vi "TDMS Initialization and Tag Formation_MS.vi"(8 "error in":errorcluster caption="エラー入力（エラーなし）", 10 "Raw data":dbl[](array[numeric]), 11 "A TDMS Pass":path) -> (0 "error out":errorcluster caption="エラー出力", 2 "Table Tag C":T1, 3 "A TDMSファイル出力":refnum<k34>)   [LabVIEW 2018]
panel:
  out "AC Table Tag":string[](array[string])
  out "AR Table Tag":string[](array[string])
  out "B Table Tag":string[](array[string])
  out "R Table Tag":string[](array[string])
  out "S Table Tag":string[](array[string])
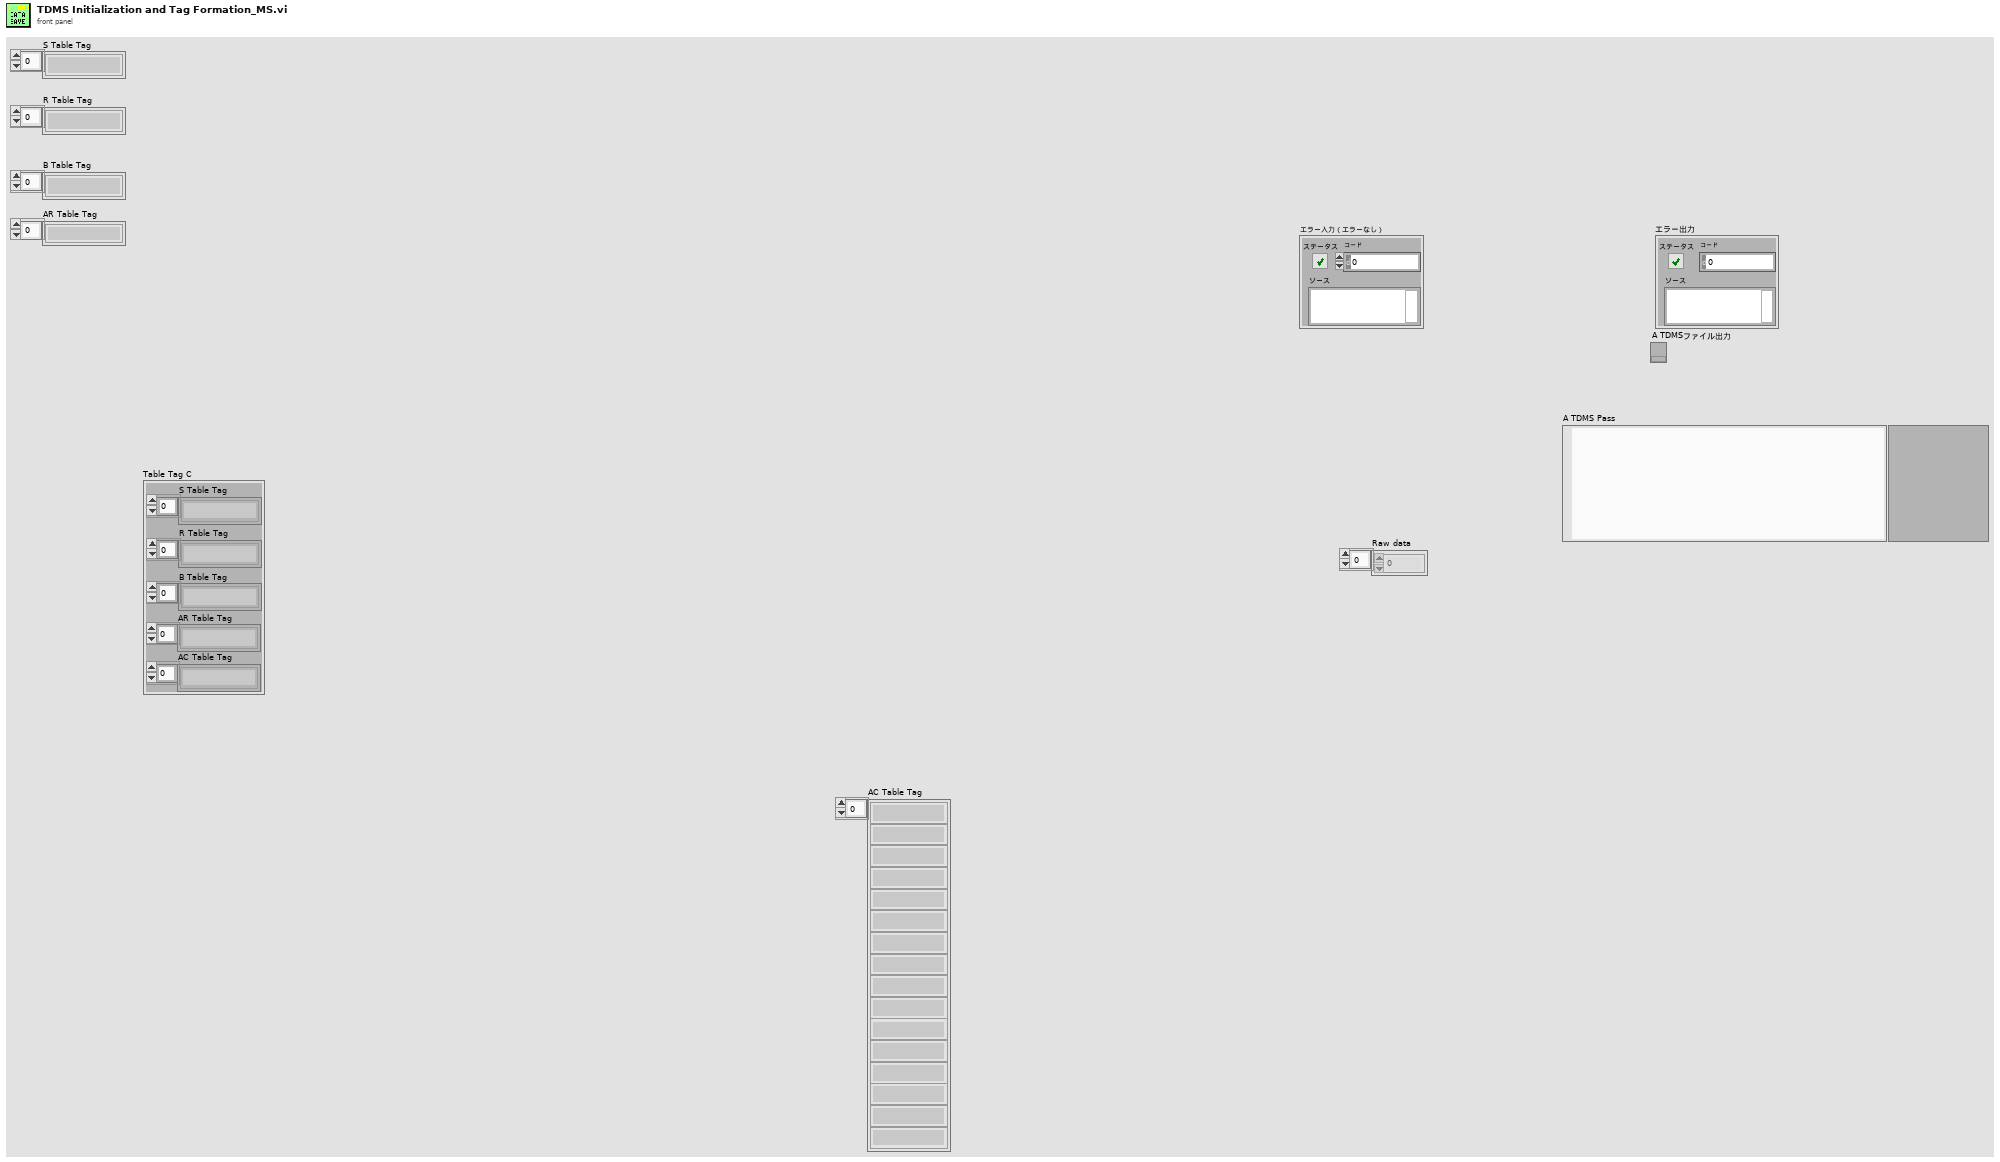
[diagram p1: front panel]
types:
  T1 = cluster{"S Table Tag":string[], "R Table Tag":string[], "B Table Tag":string[], "AR Table Tag":string[], "AC Table Tag":string[]}
  T2 = enum16{"open", "open or create", "create or replace", "create", "open (read-only)"}
  T3 = cluster{"行ヘッダ文字列[]":string[], "行ヘッダ文字列[]":string[], "行ヘッダ文字列[]":string[], "行ヘッダ文字列[]":string[], "行ヘッダ文字列[]":string[]}
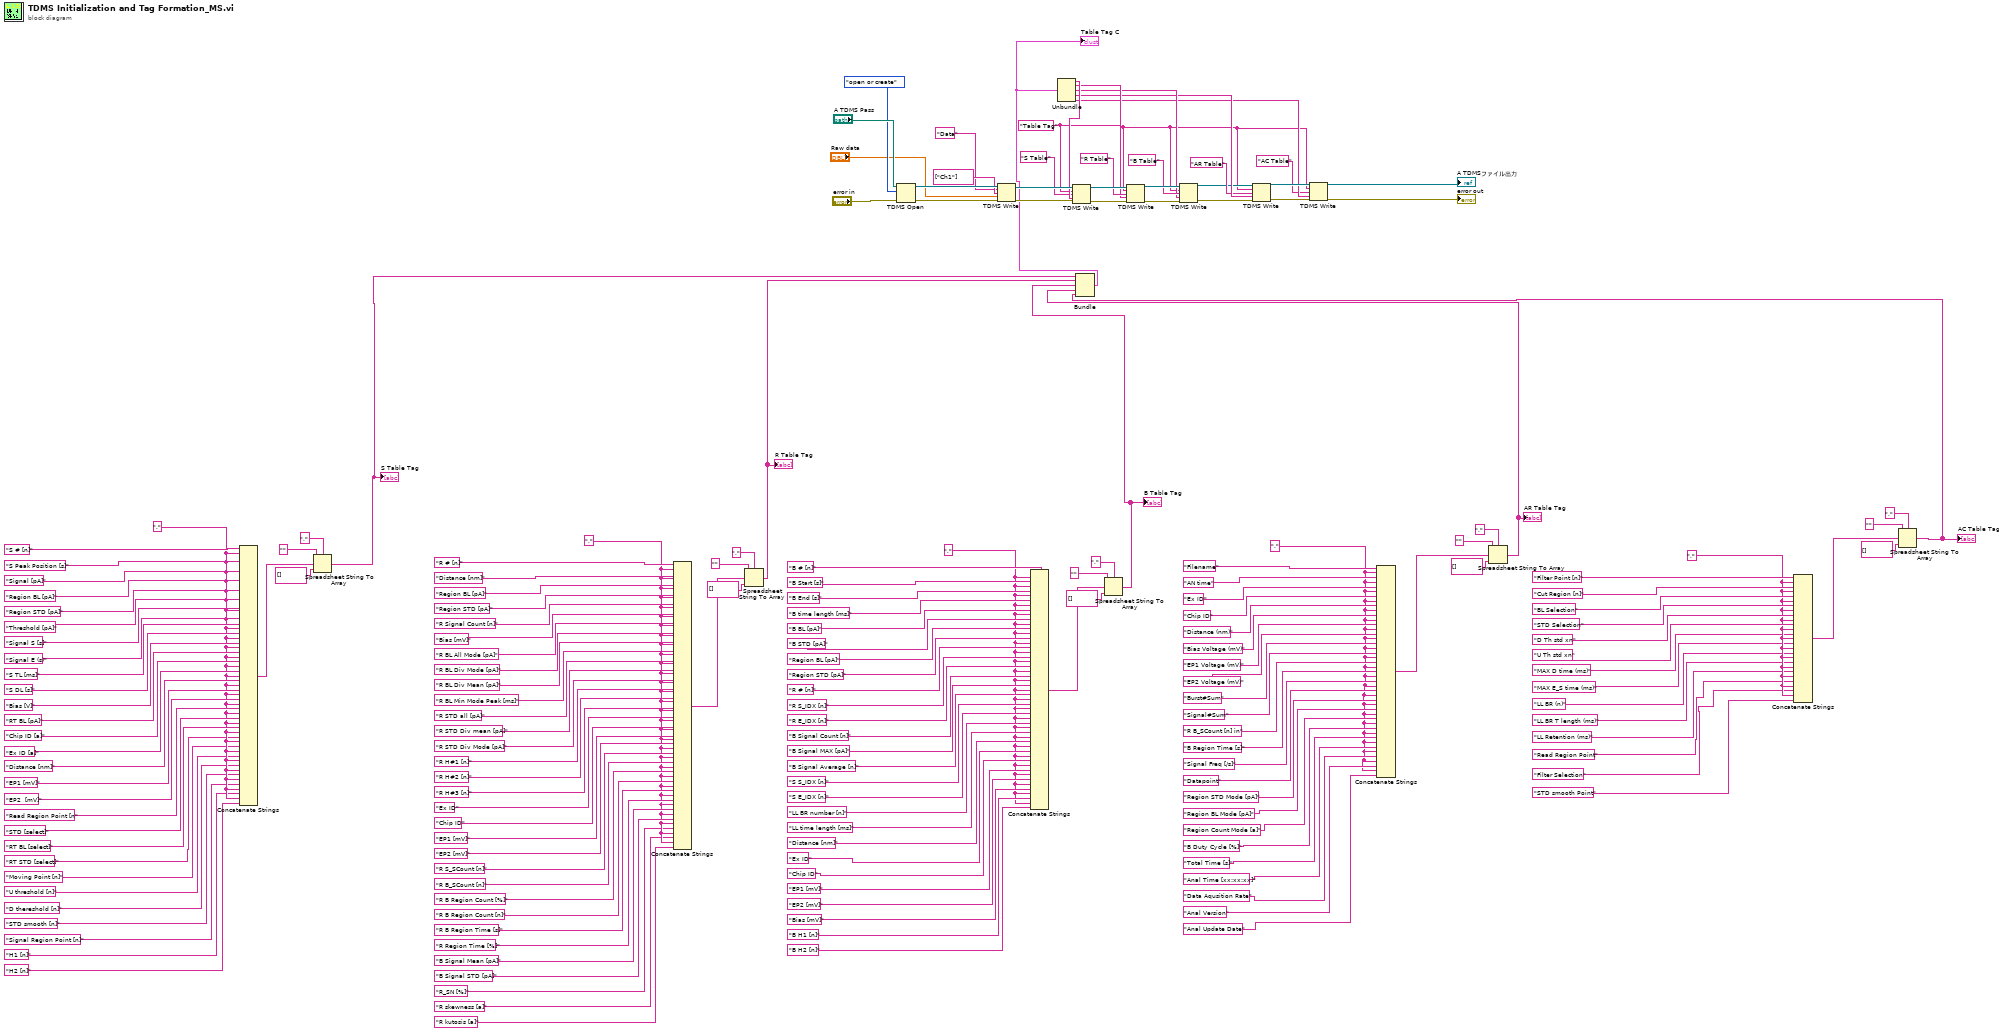
[diagram p0: block diagram]
diagram:
  w17 = "," ("デリミタ（タブ）")
  w37 = "," ("デリミタ（タブ）")
  w67 = "," ("デリミタ（タブ）")
  w105 = "," ("デリミタ（タブ）")
  w131 = "," ("デリミタ（タブ）")
  w1 = "Table Tag" ("グループ名入力（名称未設定）")
  n1 = Concatenate Strings("S # [n]" ("文字列"), w105, "S Peak Position [s]" ("文字列"), w105, "Signal [pA]" ("文字列"), w105, "Region BL [pA]" ("文字列"), w105, "Region STD [pA]" ("文字列"), w105, "Threshold [pA]" ("文字列"), w105, "Signal S [s]" ("文字列"), w105, "Signal E (s)" ("文字列"), w105, "S TL [ms]" ("文字列"), w105, "S DL [s]" ("文字列"), w105, "Bias [V]" ("文字列"), w105, "RT BL [pA]" ("文字列"), w105, "Chip ID [a]" ("文字列"), w105, "Ex ID [a]" ("文字列"), w105, "Distance [nm]" ("文字列"), w105, "EP1 [mV]" ("文字列"), w105, "EP2  [mV]" ("文字列"), w105, "Read Region Point [n" ("文字列"), w105, "STD [select]" ("文字列"), w105, "RT BL [select]" ("文字列"), w105, "RT STD [select]" ("文字列"), w105, "Moving Point [n]" ("文字列"), w105, "U threshold [n]" ("文字列"), w105, "D thereshold [n]" ("文字列"), w105, "STD smooth [n]" ("文字列"), w105, "Signal Region Point [n]" ("文字列"), w105, "H1 [n]" ("文字列"), w105, "H2 [n]" ("文字列")) -> (w125:string)
  n2 = Spreadsheet String To Array(delimiter (Tab)="," ("デリミタ（タブ）"), format string="" ("形式文字列"), spreadsheet string=w125, array type (2D Dbl)=string[] [] ("行ヘッダ文字列[]")) -> (array=w35:string[])
  "S Table Tag" <- w35
  n3 = Concatenate Strings("R # [n]" ("文字列"), w131, "Distance [nm]" ("文字列"), w131, "Region BL [pA]" ("文字列"), w131, "Region STD [pA]" ("文字列"), w131, "R Signal Count [n]" ("文字列"), w131, "Bias [mV]" ("文字列"), w131, "R BL All Mode [pA]" ("文字列"), w131, "R BL Div Mode [pA]" ("文字列"), w131, "R BL Div Mean [pA]" ("文字列"), w131, "R BL Min Mode Peak [ms]" ("文字列"), w131, "R STD all [pA]" ("文字列"), w131, "R STD Div mean [pA]" ("文字列"), w131, "R STD Div Mode [pA]" ("文字列"), w131, "R H#1 [n]" ("文字列"), w131, "R H#2 [n]" ("文字列"), w131, "R H#3 [n]" ("文字列"), w131, "Ex ID" ("文字列"), w131, "Chip ID" ("文字列"), w131, "EP1 [mV]" ("文字列"), w131, "EP2 [mV]" ("文字列"), w131, "R S_SCount [n]" ("文字列"), w131, "R B_SCount [n]" ("文字列"), w131, "R B Region Count [%]" ("文字列"), w131, "R B Region Count [n]" ("文字列"), w131, "R B Region Time [s]" ("文字列"), w131, "R Region Time [%]" ("文字列"), w131, "B Signal Mean [pA]" ("文字列"), w131, "B Signal STD [pA]" ("文字列"), w131, "R_SN [%]" ("文字列"), w131, "R skewness [a]" ("文字列"), w131, "R kutosis [a]" ("文字列")) -> (w160:string)
  n4 = Spreadsheet String To Array(delimiter (Tab)="," ("デリミタ（タブ）"), format string="" ("形式文字列"), spreadsheet string=w160, array type (2D Dbl)=string[] [] ("行ヘッダ文字列[]")) -> (array=w34:string[])
  "R Table Tag" <- w34
  n5 = TDMS Open(8:"error in", 10:T2."open or create" ("操作（0:open）"), 11:"A TDMS Pass") -> (0:w181:errorcluster, 3:w180:refnum<k34>)  [unwired: 4 in]
  n6 = TDMS Write(0:w180, 5:"Data" ("グループ名入力（名称未設定）"), 7:string[] ["Ch1"] ("チャンネル名入力（名称未設定）"), 9:"Raw data", 11:w181) -> (4:w175:refnum<k34>, 15:w176:errorcluster)  [unwired: 1 in, 2 out]
  n7 = Concatenate Strings("B # [n]" ("文字列"), w67, "B Start [s]" ("文字列"), w67, "B End [s]" ("文字列"), w67, "B time length [ms]" ("文字列"), w67, "B BL [pA]" ("文字列"), w67, "B STD [pA]" ("文字列"), w67, "Region BL [pA]" ("文字列"), w67, "Region STD [pA]" ("文字列"), w67, "R # [n]" ("文字列"), w67, "R S_IDX [n]" ("文字列"), w67, "R E_IDX [n]" ("文字列"), w67, "B Signal Count [n]" ("文字列"), w67, "B Signal MAX [pA]" ("文字列"), w67, "B Signal Average [n]" ("文字列"), w67, "S S_IDX [n]" ("文字列"), w67, "S E_IDX [n]" ("文字列"), w67, "LL BR number [n]" ("文字列"), w67, "LL time length [ms]" ("文字列"), w67, "Distance [nm]" ("文字列"), w67, "Ex ID" ("文字列"), w67, "Chip ID" ("文字列"), w67, "EP1 [mV]" ("文字列"), w67, "EP2 [mV]" ("文字列"), w67, "Bias [mV]" ("文字列"), w67, "B H1 [n]" ("文字列"), w67, "B H2 [n]" ("文字列")) -> (w92:string)
  n8 = Spreadsheet String To Array(delimiter (Tab)="," ("デリミタ（タブ）"), format string="" ("形式文字列"), spreadsheet string=w92, array type (2D Dbl)=string[] [] ("行ヘッダ文字列[]")) -> (array=w64:string[])
  "B Table Tag" <- w64
  n9 = Concatenate Strings("Filename" ("文字列"), w37, "AN time" ("文字列"), w37, "Ex ID" ("文字列"), w37, "Chip ID" ("文字列"), w37, "Distance (nm)" ("文字列"), w37, "Bias Voltage (mV)" ("文字列"), w37, "EP1 Voltage (mV)" ("文字列"), w37, "EP2 Voltage (mV)" ("文字列"), w37, "Burst#Sum" ("文字列"), w37, "Signal#Sum" ("文字列"), w37, "R B_SCount [n] in" ("文字列"), w37, "B Region Time [s]" ("文字列"), w37, "Signal Freq [/s]" ("文字列"), w37, "Datapoint" ("文字列"), w37, "Region STD Mode [pA]" ("文字列"), w37, "Region BL Mode [pA]" ("文字列"), w37, "Region Count Mode [a]" ("文字列"), w37, "B Duty Cycle [%]" ("文字列"), w37, "Total Time [s]" ("文字列"), w37, "Anal Time [xx:xx:xx]" ("文字列"), w37, "Data Aqusition Rate" ("文字列"), w37, "Anal Version" ("文字列"), w37, "Anal Update Date" ("文字列")) -> (w59:string)
  n10 = Spreadsheet String To Array(delimiter (Tab)="," ("デリミタ（タブ）"), format string="" ("形式文字列"), spreadsheet string=w59, array type (2D Dbl)=string[] [] ("行ヘッダ文字列[]")) -> (array=w33:string[])
  "AR Table Tag" <- w33
  n11 = Concatenate Strings("Filter Point [n]" ("文字列"), w17, "Cut Region [n]" ("文字列"), w17, "BL Selection" ("文字列"), w17, "STD Selection" ("文字列"), w17, "D Th std xn" ("文字列"), w17, "U Th std xn" ("文字列"), w17, "MAX D time (ms)" ("文字列"), w17, "MAX E_S time (ms)" ("文字列"), w17, "LL BR (n)" ("文字列"), w17, "LL BR T length (ms)" ("文字列"), w17, "LL Retention (ms)" ("文字列"), w17, "Read Region Point" ("文字列"), w17, "Filter Selection" ("文字列"), w17, "STD smooth Point" ("文字列")) -> (w23:string)
  n12 = Spreadsheet String To Array(delimiter (Tab)="," ("デリミタ（タブ）"), format string="" ("形式文字列"), spreadsheet string=w23, array type (2D Dbl)=string[] [] ("行ヘッダ文字列[]")) -> (array=w8:string[])
  "AC Table Tag" <- w8
  n13 = Bundle("行ヘッダ文字列[]"=w35, "行ヘッダ文字列[]"=w34, "行ヘッダ文字列[]"=w64, "行ヘッダ文字列[]"=w33, "行ヘッダ文字列[]"=w8) -> (w32:T3)  [unwired: 1 in]
  "Table Tag C" <- w32
  n14 = Unbundle(w32) -> ("行ヘッダ文字列[]"=w170:string[], "行ヘッダ文字列[]"=w167:string[], "行ヘッダ文字列[]"=w165:string[], "行ヘッダ文字列[]"=w30:string[], "行ヘッダ文字列[]"=w3:string[])
  n15 = TDMS Write(0:w175, 5:w1, 7:"S Table" ("チャンネル名入力（名称未設定）"), 9:w170, 11:w176) -> (4:w172:refnum<k34>, 15:w174:errorcluster)  [unwired: 1 in, 2 out]
  n16 = TDMS Write(0:w172, 5:w1, 7:"R Table" ("チャンネル名入力（名称未設定）"), 9:w167, 11:w174) -> (4:w171:refnum<k34>, 15:w173:errorcluster)  [unwired: 1 in, 2 out]
  n17 = TDMS Write(0:w171, 5:w1, 7:"B Table" ("チャンネル名入力（名称未設定）"), 9:w165, 11:w173) -> (4:w28:refnum<k34>, 15:w31:errorcluster)  [unwired: 1 in, 2 out]
  n18 = TDMS Write(0:w28, 5:w1, 7:"AR Table" ("チャンネル名入力（名称未設定）"), 9:w30, 11:w31) -> (4:w7:refnum<k34>, 15:w5:errorcluster)  [unwired: 1 in, 2 out]
  n19 = TDMS Write(0:w7, 5:w1, 7:"AC Table" ("Group name"), 9:w3, 11:w5) -> (4:→"A TDMSファイル出力":refnum<k34>, 15:→"error out":errorcluster)  [unwired: 1 in, 2 out]
